vi "B_ASD Signal Assignment VI.vi"(8 "BR End time (s)":dbl, 9 "BR Start time (s)":dbl, 11 "Under D array":T2) -> (3 "Under D B Array":T1)   [LabVIEW 2018]
panel:
  out "BR I-t profie":cluster{dbl[], dbl[]}(graph)
  out "B Under D IDX":i32[](array[numeric])
  out "B Under D Signal":dbl[](array[numeric])
  out "B Under D Time":dbl[](array[numeric])
  out "サイズ":i32
  out "Under D Signal":dbl[](array[numeric])
  out "Under D time":dbl[](array[numeric])
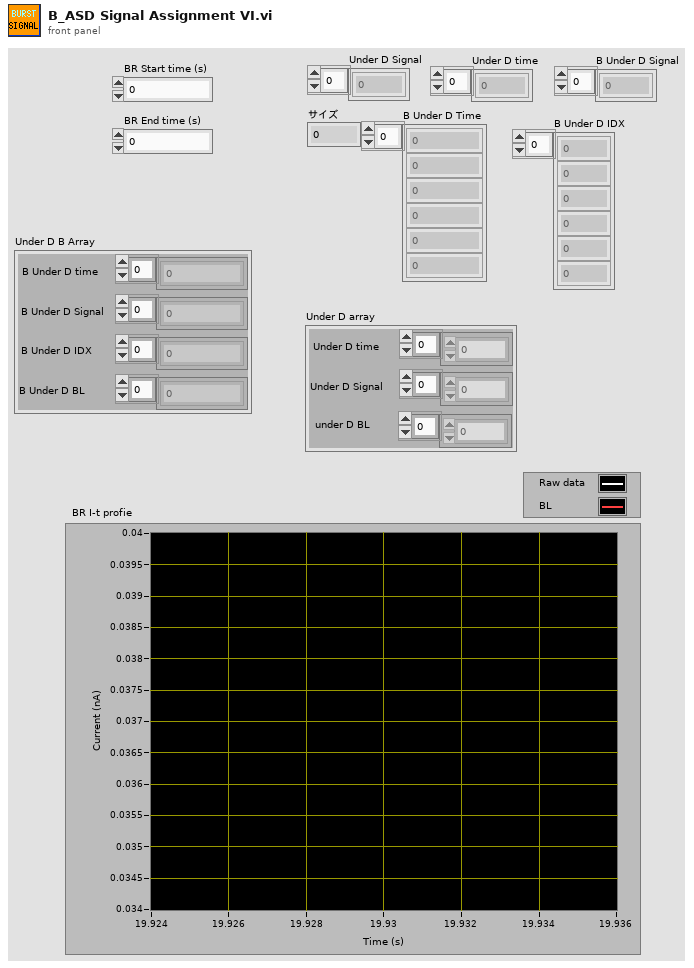
[diagram p1: front panel]
types:
  T1 = cluster{"B Under D time":dbl[], "B Under D Signal ":dbl[], "B Under D IDX":i32[], "B Under D BL":dbl[]}
  T2 = cluster{"Under D time":dbl[], "Under D Signal":dbl[], "under D BL":dbl[]}
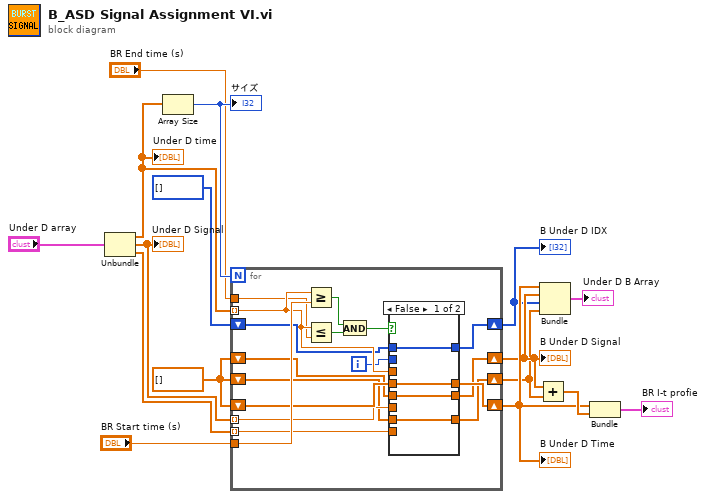
[diagram p0: block diagram]
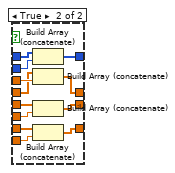
[diagram p2: hidden frame]
diagram:
  w7 = dbl[] []
  n1 = Unbundle("Under D array") -> ("Under D time"=w15:dbl[], "Under D Signal"=w11:dbl[], "under D BL"=w8:dbl[])
  "Under D time" <- w15
  "Under D Signal" <- w11
  n2 = Array Size(array=w15) -> (size(s)=w16:i32)
  "サイズ" <- w16
  n3 = for {
    N: w16 -> [_]
    tunnel: w15 -> [w29] mode=indexing
    tunnel: "BR Start time (s)" -> [w33]
    tunnel: "BR End time (s)" -> [w26]
    shift-right: [w28] -> w5
    shift-left: w7 -> [w27]
    shift-right: [w25] -> w4
    shift-left: w7 -> [w24]
    shift-right: [w22] -> w3
    shift-left: i32[] [] -> [w21]
    tunnel: w11 -> [w20] mode=indexing
    tunnel: w8 -> [w19] mode=indexing
    shift-right: [w18] -> w2
    shift-left: w7 -> [w17]
    i -> [w23]
    n4 = Greater Or Equal?(x=w29, y=w33) -> (x >= y?=w32:bool)
    n5 = Less Or Equal?(x=w29, y=w26) -> (x <= y?=w31:bool)
    n6 = And(x=w32, y=w31) -> (x .and. y?=w30:bool)
    n7 = case shown="False" w30 {
      tunnel: w29 -> [_ w49]
      tunnel: [w37 w48] -> w28
      tunnel: w27 -> [w37 w47]
      tunnel: w20 -> [_ w46]
      tunnel: [w36 w45] -> w25
      tunnel: w24 -> [w36 w44]
      tunnel: w23 -> [_ w43]
      tunnel: [w35 w42] -> w22
      tunnel: w21 -> [w35 w41]
      tunnel: w19 -> [_ w40]
      tunnel: [w34 w39] -> w18
      tunnel: w17 -> [w34 w38]
      frame False {
      }
      frame True {
        n8 = Build Array (concatenate)(w41, w43) -> (w42:i32[])
        n9 = Build Array (concatenate)(w47, w49) -> (w48:dbl[])
        n10 = Build Array (concatenate)(w44, w46) -> (w45:dbl[])
        n11 = Build Array (concatenate)(w38, w40) -> (w39:dbl[])
      }
    }
  }
  "B Under D Time" <- w5
  "B Under D Signal" <- w4
  "B Under D IDX" <- w3
  n12 = Add(x=w4, y=w2) -> (x+y=w6:dbl[])
  n13 = Bundle(w5, w4, w3, w2) -> (→"Under D B Array":cluster{dbl[], dbl[], i32[], dbl[]})  [unwired: 1 in]
  n14 = Bundle(w5, w6) -> (→"BR I-t profie":cluster{dbl[], dbl[]})  [unwired: 1 in]
